vi "Add String to Array Constant.vi"(8 "error in":errorcluster, 9 "New Value":string, 10 "Array Constant Label":string, 11 "VI Ref in":refnum<vi>) -> (0 "error out":errorcluster, 3 "VI Ref out":refnum<vi>)   [LabVIEW 2026]
doc: "Add a string element to an array of strings constant."
uses:
  <vilib>/Utility/traverseref.llb/TRef TravTarget.ctl
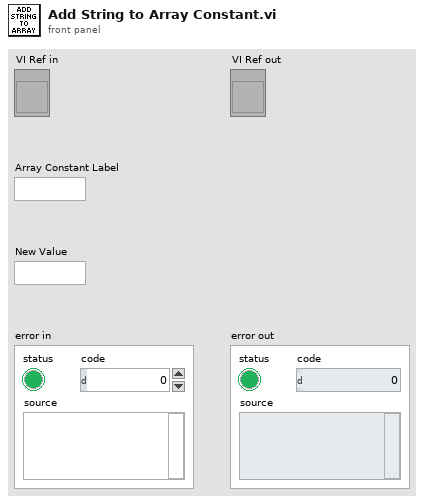
[diagram p1: front panel]
types:
  T1 = typedef "TRef TravTarget.ctl" = enum16{"FP", "BD", "Other"}
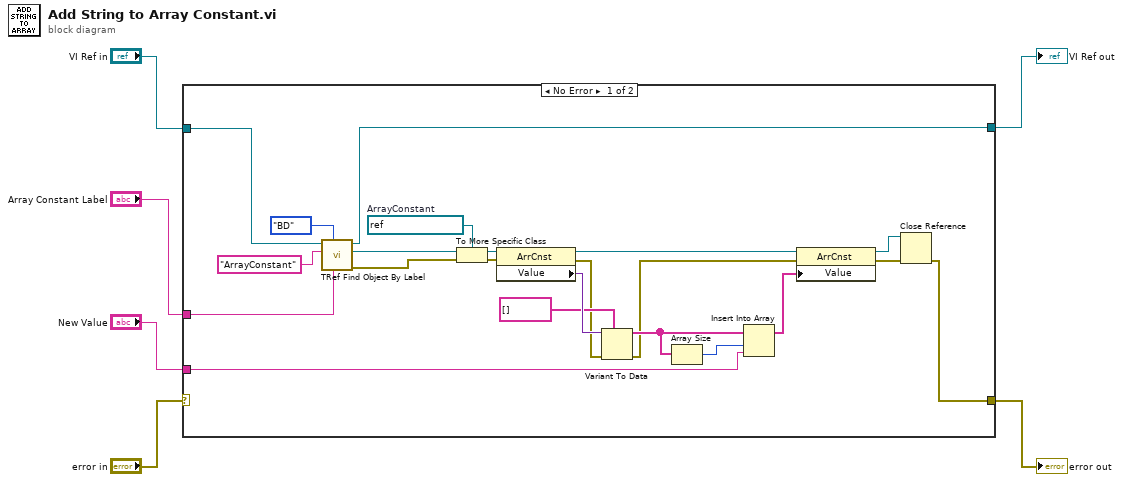
[diagram p0: block diagram]
diagram:
  n1 = case shown="No Error" "error in" {
    selector: "error in" -> [_ w30]
    tunnel: "VI Ref in" -> [w11 w29]
    tunnel: [w10 w29] -> w5
    tunnel: "Array Constant Label" -> [w9 _]
    tunnel: "New Value" -> [w8 _]
    tunnel: [w7 w30] -> w2
    frame No Error {
      w24 = refnum<vi> refnum  # ArrayConstant
      n2 = call <vilib>:"TRef Find Object By Label.vi"("Label"=w9, "Traverse Target"=TRef_TravTarget."BD", "Class Name"="ArrayConstant", "VI Ref"=w11) -> ("error out"=w25:errorcluster, "Found Obj Ref"=w26:refnum<vi>, "dup VI Ref"=w10:refnum<vi>)  [unwired: 4 in, 1 out]
      n3 = To More Specific Class(target class=w24, reference=w26, error in=w25) -> (specific class reference=w23:refnum<vi>, error out=w21:errorcluster)
      n4 = property class="ArrCnst"(reference=w23, error in=w21) -> (reference out=w22:refnum<vi>, error out=w18:errorcluster, "Value"=w20:variant)
      n5 = Variant To Data(error in=w18, type=string[] [], Variant=w20) -> (data=w17:string[], error out=w14:errorcluster)
      n6 = Array Size(array=w17) -> (size(s)=w16:i32)
      n7 = Insert Into Array(array=w17, index=w16, new element=w8) -> (w15:string[])
      n8 = property class="ArrCnst"(reference=w22, error in=w14, "Value"=w15) -> (reference out=w12:refnum<vi>, error out=w13:errorcluster)
      n9 = Close Reference(reference=w12, error in (no error)=w13) -> (error out=w7:errorcluster)
    }
    frame Error {
      # "Pass error without further action."
    }
  }
  "VI Ref out" <- w5
  "error out" <- w2
